vi "Status String Update.vi"(6 "error in (no error)":errorcluster, 10 "Value":string, 11 "String reference in":refnum<vi>) -> (3 "STring reference out":refnum<vi>)   [LabVIEW 2019]
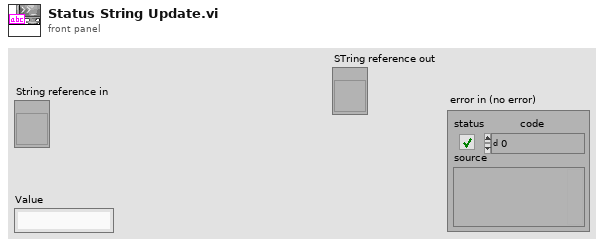
[diagram p1: front panel]
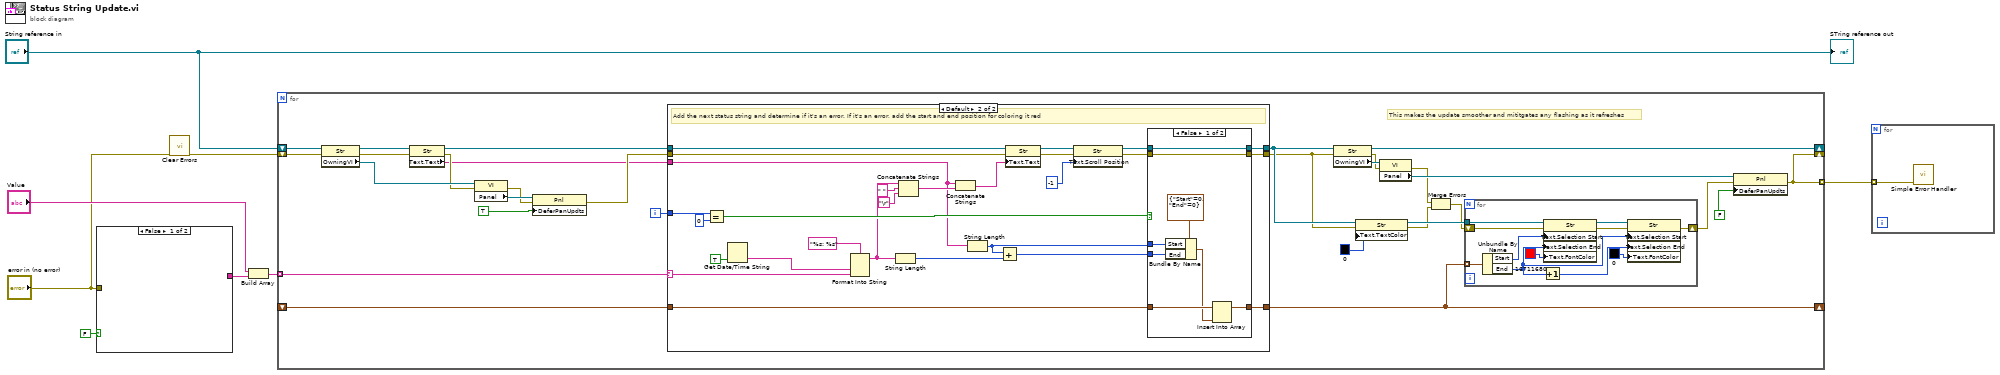
[diagram p0: block diagram]
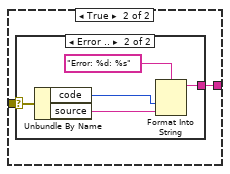
[diagram p2: hidden frame]
diagram:
  n1 = case shown="False" FALSE {
    tunnel: [_ w10] -> w6
    tunnel: "error in (no error)" -> [_ w9]
    frame False {
    }
    frame True {
      n2 = case shown="Error .." w9 {
        selector: w9 -> [_ w15]
        tunnel: [_ w12] -> w10
        frame No Error {
        }
        frame Error {
          n3 = Unbundle By Name(w15) -> ("code"=w13:i32, "source"=w14:string)
          n4 = Format Into String(format string="Error: %d: %s", w13, w14) -> (resulting string=w12:string)  [unwired: 2 in, 1 out]
        }
      }
    }
  }
  n5 = call <vilib>:"Clear Errors.vi"("error in (no error)"="error in (no error)") -> ("error out"=w3:errorcluster)  [unwired: 5 in, 1 out]
  n6 = Build Array("Value", w6) -> (w5:string[])
  n7 = for {
    tunnel: w5 -> [w45] mode=indexing
    shift-right: [w42] -> _
    shift-left: _ -> [w43]
    shift-right: [w29] -> _
    shift-left: w3 -> [w32]
    tunnel: [w29] -> w2 mode=indexing
    shift-right: [w16] -> _
    shift-left: "String reference in" -> [w35]
    i -> [w44]
    # "This makes the update smoother and mititgates any flashing as it refreshes"
    n8 = property class="Str"(reference=w35, error in=w32) -> (reference out=w21:refnum<vi>, error out=w19:errorcluster, "OwningVI"=w38:refnum<vi>)
    n9 = property class="Str"(reference=w21, error in=w19) -> (reference out=w20:refnum<vi>, error out=w18:errorcluster, "Text.Text"=w17:string)
    n10 = property class="VI"(reference=w38, error in=w18) -> (error out=w31:errorcluster, "Panel"=w37:refnum<vi>)  [unwired: 1 out]
    n11 = property class="Pnl"(reference=w37, error in=w31, "DeferPanUpdts"=TRUE ("Defer Panel Updates")) -> (error out=w34:errorcluster)  [unwired: 1 out]
    n12 = case shown="Default" w45 {
      selector: w45 -> [_ w76]
      tunnel: w20 -> [w58 w61]
      tunnel: w44 -> [_ w81]
      tunnel: w43 -> [w59 w68]
      tunnel: [w59 w67] -> w42
      tunnel: [w58 w66] -> w27
      tunnel: w34 -> [w57 w60]
      tunnel: [w57 w63] -> w22
      tunnel: w17 -> [_ w62]
      frame "" {
      }
      frame Default {
        # "Add the next status string and determine if it's an error. If it's an error, add the start and end position for coloring it red"
        n13 = Equal?(x=w81, y=0) -> (x = y?=w75:bool)
        n14 = Get Date/Time String(want seconds? (F)=TRUE) -> (time string=w84:string)  [unwired: 2 in, 1 out]
        n15 = Format Into String(format string="%s: %s", w84, w76) -> (resulting string=w74:string)  [unwired: 2 in, 1 out]
        n16 = String Length(string=w74) -> (length=w78:i32)
        n17 = Concatenate Strings(w74, " " ("string"), "\r") -> (w71:string)
        n18 = Concatenate Strings(w62, w71) -> (w70:string)
        n19 = String Length(string=w62) -> (length=w79:i32)
        n20 = Add(x=w79, y=w78) -> (x+y=w77:i32)
        n21 = property class="Str"(reference=w61, error in=w60, "Text.Text"=w70) -> (reference out=w69:refnum<vi>, error out=w65:errorcluster)
        n22 = property class="Str"(reference=w69, error in=w65, "Text.Scroll Position"=-1) -> (reference out=w82:refnum<vi>, error out=w64:errorcluster)
        n23 = case shown="False" w75 {
          tunnel: w82 -> [w89 w96]
          tunnel: w79 -> [w94 _]
          tunnel: w77 -> [w93 _]
          tunnel: w68 -> [w92 w97]
          tunnel: [w91 w97] -> w67
          tunnel: [w89 w96] -> w66
          tunnel: w64 -> [w87 w95]
          tunnel: [w87 w95] -> w63
          frame False {
            n24 = Bundle By Name(cluster=cluster{"Start":i32, "End":i32} {"Start"=0, "End"=0}, "Start"=w94, "End"=w93) -> (w90:cluster{"Start":i32, "End":i32})
            n25 = Insert Into Array(array=w92, new element=w90) -> (w91:cluster{"Start":i32, "End":i32}[])  [unwired: 1 in]
          }
          frame True {
          }
        }
      }
    }
    n26 = property class="Str"(reference=w27, error in=w22) -> (reference out=w16:refnum<vi>, error out=w30:errorcluster, "OwningVI"=w41:refnum<vi>)
    n27 = property class="Str"(reference=w27, error in=w22, "Text.TextColor"=u32 0 ("Text.Text Colors:Text Color")) -> (reference out=w26:refnum<vi>, error out=w23:errorcluster)
    n28 = property class="VI"(reference=w41, error in=w30) -> (error out=w24:errorcluster, "Panel"=w33:refnum<vi>)  [unwired: 1 out]
    n29 = Merge Errors(w24, w23) -> (w25:errorcluster)
    n30 = for {
      tunnel: w26 -> [w56]
      tunnel: w42 -> [w55] mode=indexing
      shift-right: [w46] -> w39
      shift-left: w25 -> [w48]
      n31 = Unbundle By Name(w55) -> ("Start"=w54:i32, "End"=w49:i32)
      n32 = Increment(x=w49) -> (x+1=w52:i32)
      n33 = property class="Str"(reference=w56, error in=w48, "Text.Selection Start"=w54, "Text.Selection End"=w49, "Text.FontColor"=u32 16711680 ("Text.Font:Color")) -> (reference out=w50:refnum<vi>, error out=w47:errorcluster)
      n34 = property class="Str"(reference=w50, error in=w47, "Text.Selection Start"=w49, "Text.Selection End"=w52, "Text.FontColor"=u32 0 ("Text.Font:Color")) -> (error out=w46:errorcluster)  [unwired: 1 out]
    }
    n35 = property class="Pnl"(reference=w33, error in=w39, "DeferPanUpdts"=FALSE ("Defer Panel Updates")) -> (error out=w29:errorcluster)  [unwired: 1 out]
  }
  n36 = for {
    tunnel: w2 -> [w98] mode=indexing
    n37 = call <vilib>:"Simple Error Handler.vi"("error in (no error)"=w98) -> ()  [unwired: 4 in, 5 out]
  }
  "STring reference out" <- "String reference in"
